vi "find or create stream channel.vi"(9 "channel tags":cluster{"key":string, "value":string}[](array[cluster]), 10 "channel name":string, 11 "stream session":refnum<data-value>) -> (0 "error out":errorcluster, 3 "Channel":refnum<class "Channel.lvclass">)   [LabVIEW 2020, in "nominal core steps.lvlib"]
doc: "In the provided stream session, register a channel by name. Tags can only be set on creation and are part of the unique identification of a channel, but are not required.\n\nExamples:\nCall with \"name\", <no tags>; Call with \"name\", <no tags> => one channel\nCall with \"name\", <no tags>; Call with \"name\", tags: [sn: 123] => two channels\nCall with \"name\", tags: [sn: 123]; Call with \"name\", tags: [sn: 321] => two channels"
uses:
  nominal core steps.lvlib
  stream session.ctl
  <vilib>/Nominal/Nominal IO Client/submodules/nominal-streaming-labview-ffi/lv_src/Stream/Stream.lvclass
  channel uid.ctl
  <vilib>/Nominal/Nominal IO Client/submodules/nominal-streaming-labview-ffi/lv_src/Channel/Channel.lvclass
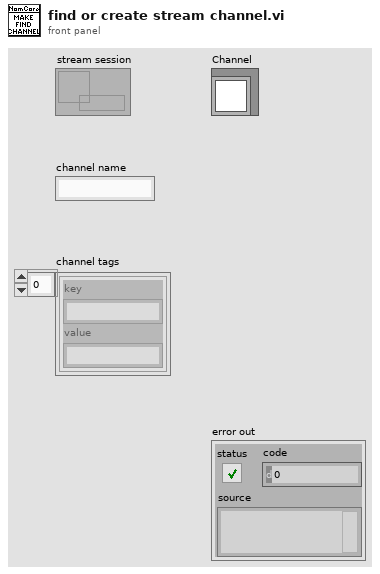
[diagram p1: front panel]
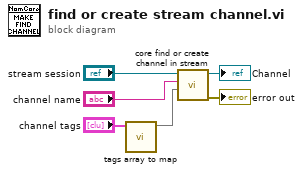
[diagram p0: block diagram]
diagram:
  n1 = call "tags array to map.vi"("channel tags"="channel tags") -> ("map"=w1:map{string, string})  [unwired: 10 in]
  n2 = call "core find or create channel in stream.vi"("tags"=w1, "channel name"="channel name", "stream"="stream session") -> ("error out"=→"error out":errorcluster, "channel"=→"Channel":refnum<class "Channel.lvclass">)  [unwired: 7 in]
